vi "Assert Not Equal Type_Variant.vi"(4 "Execution time (s)":dbl=-1.0, 5 "Assert Only? (F)":bool, 6 "error code (1)":i32=1, 7 "Label":string, 8 "error in (no error)":errorcluster, 9 "Register with caller test (F)":bool, 10 "Actual":variant, 11 "Expected":variant) -> (0 "error out":errorcluster, 2 "Properties.Assert":refnum<class "Properties.Assert.lvclass">)   [LabVIEW 2013, in "Caraya.lvlib" / "Assert.lvclass"]
doc: "Generates an error if the input condition is not met.\n\nThis method compares the value of the inputs, irrespective of the type representation.\nAsserts TRUE if input values are equal.\nAsserts FALSE otherwise.\n\nex: Two integer inputs of equal value but of different type representation (U8 and I32) will assert TRUE."
uses:
  Assert.lvclass
  Properties.Assert/Properties.Assert.lvclass
  <vilib>/Utility/VariantDataType/VariantType.lvlib
  Properties/Properties.lvclass
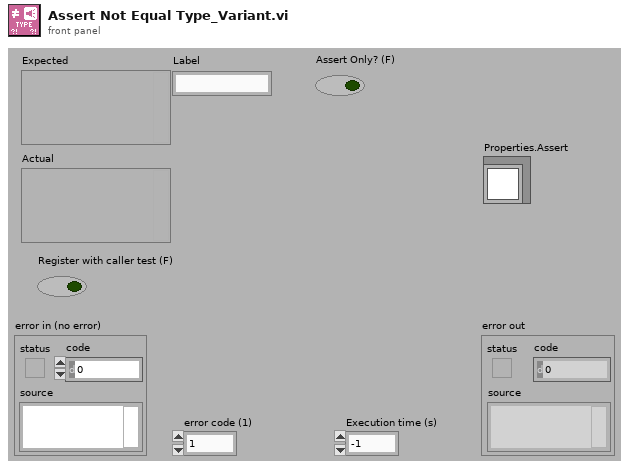
[diagram p1: front panel]
types:
  T1 = typedef "VariantType.lvlib/Type.ctl" = enum8{"Invalid Type", "Void", "I8", "I16", "I32", "I64", "U8", "U16", "U32", "U64", "Single Float", "Double Float", "Extended Float", "Single Complex", "Double Complex", "Extended Complex", "Enum U8", "Enum U16", "Enum U32", "Enum U64", "Single Float With Unit", "Double Float With Unit", "Extended Float With Unit", "Single Complex with Unit", "Double Complex with Unit", "Extended Complex with Unit", "Boolean", "String", "Path", "Picture", "Tag", "Array", "Cluster", "Variant", "LV Variant", "Waveform", "Timestamp", "Digital Waveform", "Digital Data", "ExpressData", "Refnum", "External Data", "VI", "Poly VI", "LabVIEW Class Instance", "Fixed Point"}
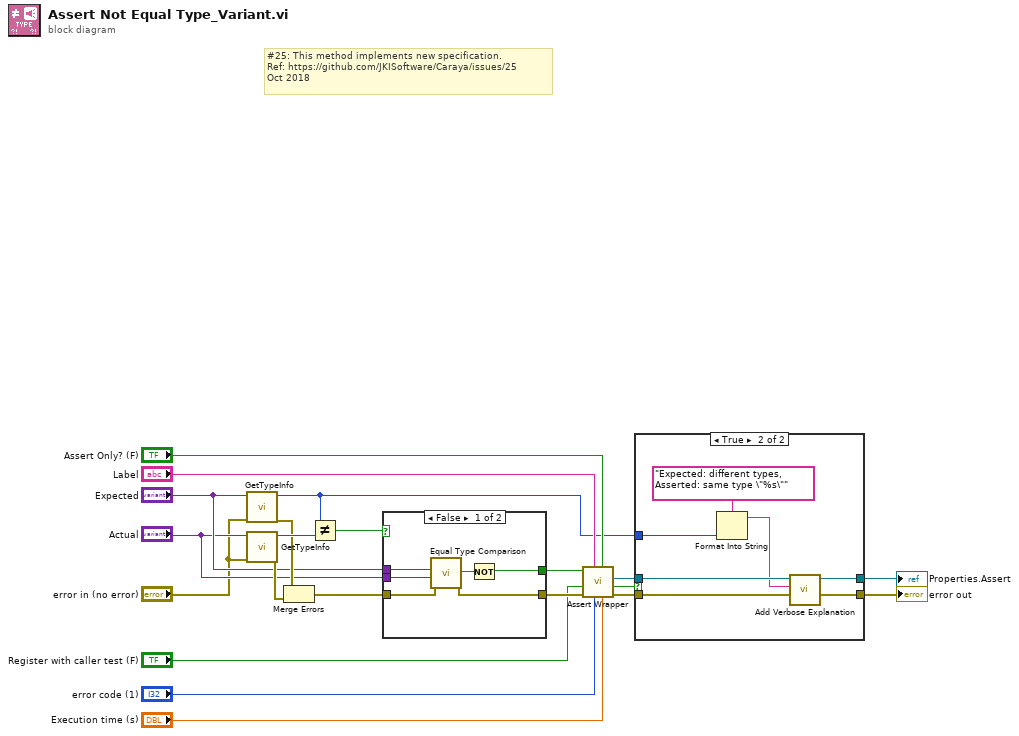
[diagram p0: block diagram]
diagram:
  # "#25: This method implements new specification.\nRef: https://github.com/JKISoftware/Caraya/issues/25\nOct 2018"
  n1 = call <vilib>:"GetTypeInfo.vi"("error in (no error)"="error in (no error)", "Variant"="Expected") -> ("error out"=w17:errorcluster, "Type Enum"=w4:T1)  [unwired: 5 in, 3 out]
  n2 = call <vilib>:"GetTypeInfo.vi"("error in (no error)"="error in (no error)", "Variant"="Actual") -> ("error out"=w16:errorcluster, "Type Enum"=w18:T1)  [unwired: 5 in, 3 out]
  n3 = Merge Errors(w17, w16) -> (w12:errorcluster)
  n4 = Not Equal?(x=w4, y=w18) -> (x != y?=w15:bool)
  n5 = case shown="False" w15 {
    selector: w15 -> [_ w29]
    tunnel: "Expected" -> [w23 _]
    tunnel: "Actual" -> [w22 _]
    tunnel: w12 -> [w27 w28]
    tunnel: [w25 w29] -> w11
    tunnel: [w24 w28] -> w10
    frame False {
      n6 = call "Equal Type Comparison.vi"("error in (no error)"=w27, "Actual"=w22, "Expected"=w23) -> ("error out"=w24:errorcluster, "Equal Types?"=w26:bool)  [unwired: 6 in, 1 out]
      n7 = Not(x=w26) -> (.not. x?=w25:bool)
    }
    frame True {
    }
  }
  n8 = call "Assert Wrapper.vi"("Execution time (s)"="Execution time (s)", "Assert Only? (F)"="Assert Only? (F)", "error code (1)"="error code (1)", "Label"="Label", "error in (no error)"=w10, "Register with caller test (F)"="Register with caller test (F)", "Assert?"=w11) -> ("error out"=w8:errorcluster, "Verbose"=w5:bool, "Properties.Assert"=w2:refnum<class "Properties.Assert.lvclass">)  [unwired: 1 in, 1 out]
  n9 = case shown="True" w5 {
    tunnel: [w31 w33] -> w7
    tunnel: w8 -> [w31 w35]
    tunnel: w4 -> [_ w38]
    tunnel: w2 -> [w30 w36]
    tunnel: [w30 w32] -> w1
    frame False {
    }
    frame True {
      n10 = Format Into String(format string="Expected: different types, Asserted: same type \"%s\"" ("t"), w38) -> (resulting string=w34:string)  [unwired: 2 in, 1 out]
      n11 = call "Add Verbose Explanation.vi"("error in (no error)"=w35, "Verbose Explanation"=w34, "Properties"=w36) -> ("error out"=w33:errorcluster, "Properties"=w32:refnum<class "Properties.Assert.lvclass">)  [unwired: 7 in]
    }
  }
  "error out" <- w7
  "Properties.Assert" <- w1
